vi "Get Errors Method.vi"   [LabVIEW 2020]
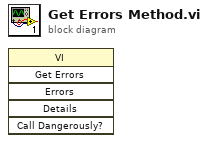
[diagram p0: block diagram]
diagram:
  n1 = invoke class="VI" method="Get Errors"() -> ()  [unwired: 6 in, 6 out]
